vi "request Call Processing Command.vi"(8 "error in (no error)":errorcluster, 10 "Call Processing Mode":T1, 11 "Anritsu Call Box_Implement in":refnum<class "Anritsu Call Box_Implement.lvclass">) -> (0 "error out":errorcluster, 3 "Anritsu Call Box_Implement out":refnum<class "Anritsu Call Box_Implement.lvclass">)   [LabVIEW 2023, in "ANRITSU Call Box.lvlib" / "Anritsu Call Box_Implement.lvclass"]
uses:
  Anritsu Call Box_Implement.lvclass
  Anritsu Call Box_Implement.lvclass/Anritsu Call Box_Implement.ctl
  LTE/LTE.lvclass
  Type Definition/Call Processing Command.ctl
  ANRITSU Call Box.lvlib
  NR/NR.lvclass
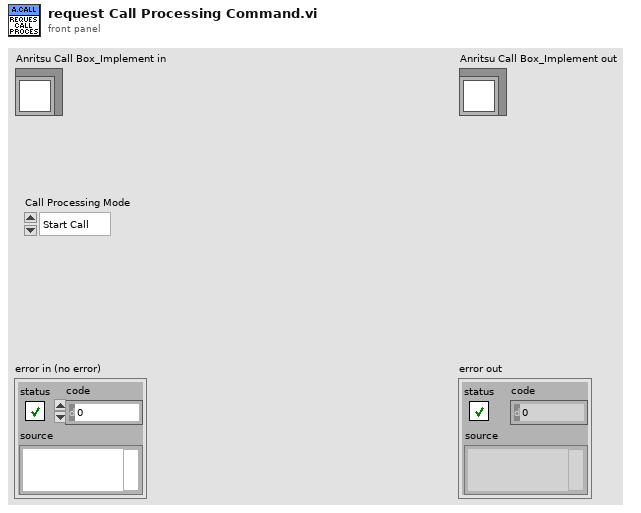
[diagram p1: front panel]
types:
  T1 = typedef "ANRITSU Call Box.lvlib/Call Processing Command.ctl" = enum16{"Start Call", "End Call"}
  T2 = typedef "ANRITSU Call Box.lvlib/Call Device - Protocol Type Selector.ctl" = enum16{"8000A - NR", "8000A - LTE", "882xC - LTE"}
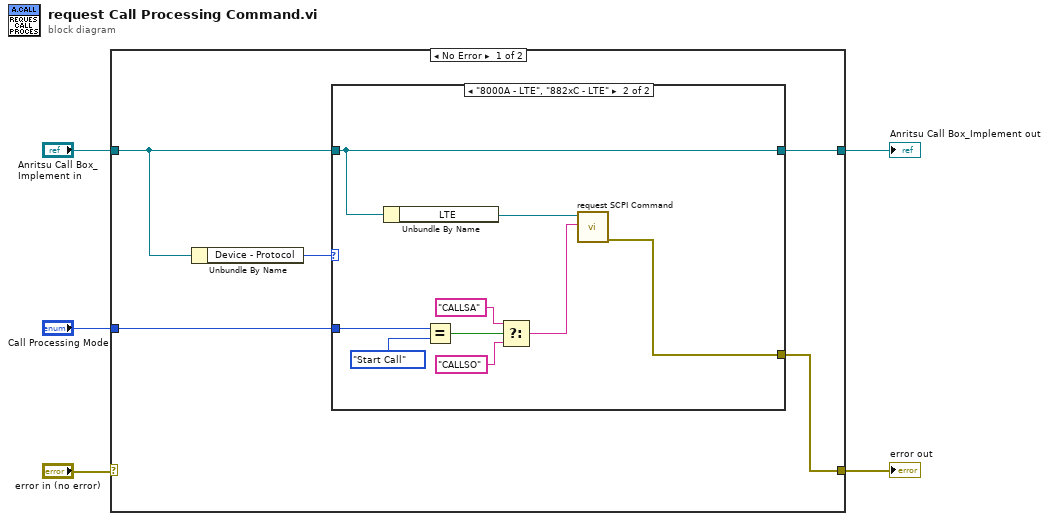
[diagram p0: block diagram]
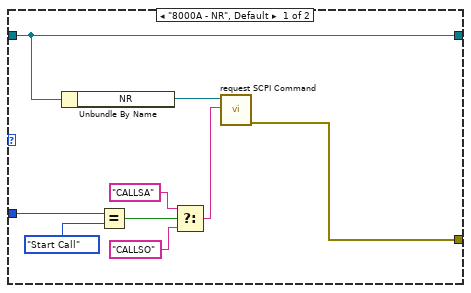
[diagram p2: hidden frame]
diagram:
  n1 = case shown="No Error" "error in (no error)" {
    selector: "error in (no error)" -> [_ w29]
    tunnel: "Anritsu Call Box_Implement in" -> [w9 w30]
    tunnel: [w8 w30] -> w4
    tunnel: [w7 w29] -> w2
    tunnel: "Call Processing Mode" -> [w6 _]
    frame No Error {
      n2 = Unbundle By Name(w9) -> ("Device - Protocol"=w10:T2)
      n3 = case shown="\"8000A - LTE\", \"882xC - LTE\"" w10 {
        tunnel: w9 -> [w19 w28]
        tunnel: [w19 w28] -> w8
        tunnel: [w11 w20] -> w7
        tunnel: w6 -> [w13 w26]
        frame "8000A - NR", Default {
          n4 = Unbundle By Name(w19) -> ("NR"=w18:refnum<class "NR.lvclass">)
          n5 = Equal?(x=w13, y=Call_Processing_Command."Start Call") -> (x = y?=w15:bool)
          n6 = Select(t="CALLSA" ("SCPI Command"), s=w15, f="CALLSO" ("SCPI Command")) -> (s? t:f=w12:string)
          n7 = call "request SCPI Command.vi"("SCPI Command"=w12, "NR in"=w18) -> ("error out"=w11:errorcluster)  [unwired: 8 in, 1 out]
        }
        frame "8000A - LTE", "882xC - LTE" {
          n8 = Unbundle By Name(w28) -> ("LTE"=w27:refnum<class "LTE.lvclass">)
          n9 = Equal?(x=w26, y=Call_Processing_Command."Start Call") -> (x = y?=w23:bool)
          n10 = Select(t="CALLSA" ("SCPI Command"), s=w23, f="CALLSO" ("SCPI Command")) -> (s? t:f=w21:string)
          n11 = call "request SCPI Command.vi"("SCPI Command"=w21, "LTE in"=w27) -> ("error out"=w20:errorcluster)  [unwired: 8 in, 1 out]
        }
      }
    }
    frame Error {
    }
  }
  "error out" <- w2
  "Anritsu Call Box_Implement out" <- w4
